vi "raise_any_errors.vi"(8 "error in (no error)":errorcluster, 11 "Request in":refnum<class "Request.lvclass">) -> (0 "error out":errorcluster, 3 "Request out":refnum<class "Request.lvclass">)   [LabVIEW 2020, in "reqwest.lvlib" / "Request.lvclass"]
uses:
  Request.lvclass
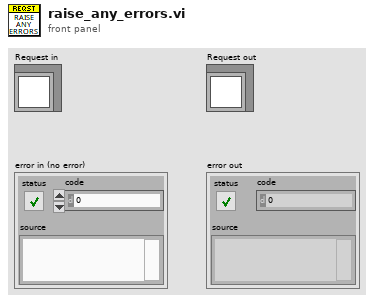
[diagram p1: front panel]
types:
  T1 = typedef "reqwest.lvlib/Request.lvclass/reqwest_error_kind_enum.ctl" = enum16{"none", "timeout", "connection", "redirect", "invalid_status", "body", "decode", "builder", "request", "file_system", "unknown"}
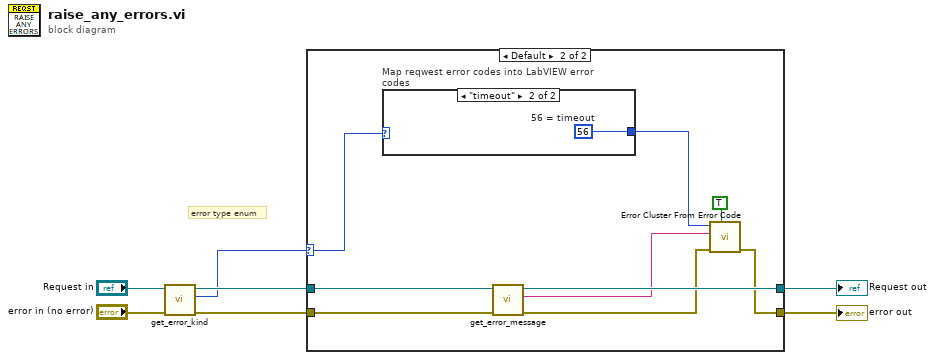
[diagram p0: block diagram]
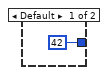
[diagram p3: hidden frame]
diagram:
  # "error type enum"
  n1 = call "get_error_kind.vi"("error in (no error)"="error in (no error)", "Request in"="Request in") -> ("error out"=w2:errorcluster, "error_kind"=w1:T1, "Request out"=w3:refnum<class "Request.lvclass">)  [unwired: 7 in]
  n2 = case shown="Default" w1 {
    selector: w1 -> [_ w11]
    tunnel: [w9 w18] -> w5
    tunnel: [w8 w17] -> w4
    tunnel: w3 -> [w9 w13]
    tunnel: w2 -> [w8 w12]
    frame "none" {
    }
    frame Default {
      n3 = case "Map reqwest error codes into LabVIEW error codes" shown="\"timeout\"" w11 {
        tunnel: [42 ("error code (0)") w20] -> w15
        frame Default {
        }
        frame "timeout" {
          w20 = 56  # 56 = timeout
        }
      }
      n4 = call "get_error_message.vi"("error in (no error)"=w12, "Request in"=w13) -> ("error out"=w16:errorcluster, "error_message"=w10:string, "Request in"=w18:refnum<class "Request.lvclass">)  [unwired: 7 in]
      n5 = call <vilib>:"Error Cluster From Error Code.vi"("show call chain? (False)"=TRUE, "error in (no error)"=w16, "error message (\"\")"=w10, "error code (0)"=w15) -> ("error out"=w17:errorcluster)  [unwired: 5 in]
    }
  }
  "Request out" <- w5
  "error out" <- w4
